vi "VIH HelpGen - Create Wrapper VI.vi"(8 "error in":errorcluster, 9 "Wrapper VI Refnum (opt)":refnum<vi>, 10 "Original VI path":path, 11 "Original VI Refnum":refnum<vi>) -> (0 "error out":errorcluster, 1 "Wrapper VI Refnum":refnum<vi>, 3 "dup Original VI Refnum":refnum<vi>)   [LabVIEW 2014]
doc: "::: VI Helpeks :::\nCopyright (c) 2000-2026 Konstantin Shifershteyn. All rights reserved."
panel:
  # "VI Helpeks\nCopyright (c) 2012-2026 Konstantin Shifershteyn"
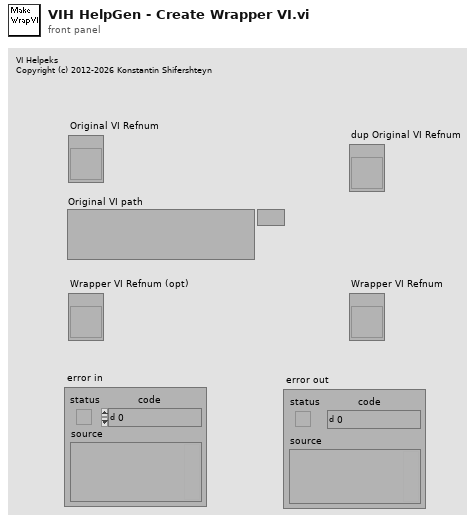
[diagram p1: front panel]
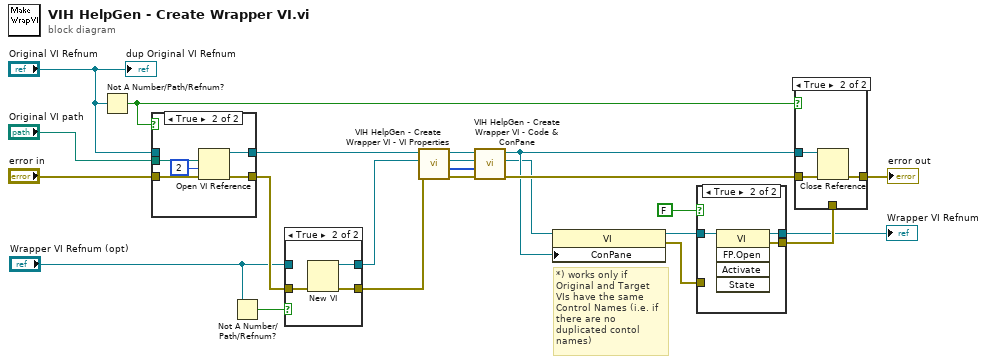
[diagram p0: block diagram]
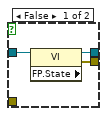
[diagram p2: hidden frame]
diagram:
  # "*) works only if Original and Target VIs have the same Control Names (i.e. if there are no duplicated contol names)"
  n1 = Not A Number/Path/Refnum?(number/path/refnum="Original VI Refnum") -> (NaN/Path/Refnum?=w13:bool)
  n2 = case shown="True" w13 {
    tunnel: "Original VI path" -> [_ w30]
    tunnel: [w25 w29] -> w22
    tunnel: [w24 w28] -> w20
    tunnel: "error in" -> [w24 w27]
    tunnel: "Original VI Refnum" -> [w25 _]
    frame False {
    }
    frame True {
      n3 = Open VI Reference(vi path=w30, options=2, error in (no error)=w27) -> (vi reference=w29:refnum<vi>, error out=w28:errorcluster)  [unwired: 3 in]
    }
  }
  n4 = Not A Number/Path/Refnum?(number/path/refnum="Wrapper VI Refnum (opt)") -> (NaN/Path/Refnum?=w10:bool)
  n5 = case shown="True" w10 {
    tunnel: w20 -> [w31 w35]
    tunnel: [w32 w34] -> w19
    tunnel: [w31 w33] -> w18
    tunnel: "Wrapper VI Refnum (opt)" -> [w32 _]
    frame False {
    }
    frame True {
      n6 = New VI(8:w35) -> (0:w33:errorcluster, 3:w34:refnum<vi>)  [unwired: 6 in]
    }
  }
  n7 = call "VIH HelpGen - Create Wrapper VI - VI Properties.vi"("error in"=w18, "Target VI Refnum"=w19, "Source VI Refnum"=w22) -> ("error out"=w21:errorcluster, "Terminal Wiring Rules"=w11:u16[], "dup Target VI Refnum"=w17:refnum<vi>, "dup Source VI Refnum"=w16:refnum<vi>)  [unwired: 5 in]
  n8 = call "VIH HelpGen - Create Wrapper VI - Code & ConPane.vi"("error in"=w21, "Terminal Wiring Rules"=w11, "Target VI Refnum"=w17, "Source VI Refnum"=w16) -> ("error out"=w12:errorcluster, "dup Target VI Refnum"=w7:refnum<vi>, "dup Source VI Refnum"=w8:refnum<vi>)  [unwired: 5 in]
  n9 = property class="VI"(reference=w7, "ConPane"=w8) -> (reference out=w6:refnum<vi>, error out=w1:errorcluster)  [unwired: 1 in]
  n10 = case shown="True" FALSE {
    tunnel: w6 -> [w38 w41]
    tunnel: [w36 w40] -> w5
    tunnel: [w37 w39] -> w4
    tunnel: w1 -> [_ _]
    frame False {
      n11 = property class="VI" props=["FP.State"](reference=w38) -> (reference out=w37:refnum<vi>, error out=w36:errorcluster)  [unwired: 1 in, 1 out]
    }
    frame True {
      n12 = invoke class="VI" method="FP.Open"(reference=w41) -> (reference out=w39:refnum<vi>, error out=w40:errorcluster)  [unwired: 4 in, 3 out]
    }
  }
  "Wrapper VI Refnum" <- w4
  n13 = case shown="True" w13 {
    tunnel: w8 -> [_ w45]
    tunnel: [w42 w44] -> w3
    tunnel: w12 -> [w42 w43]
    tunnel: w5 -> [_ _]
    frame False {
    }
    frame True {
      n14 = Close Reference(reference=w45, error in (no error)=w43) -> (error out=w44:errorcluster)
    }
  }
  "error out" <- w3
  "dup Original VI Refnum" <- "Original VI Refnum"
